vi "Close References.vi"(8 "error in":errorcluster, 11 "IProject Manager in":refnum<class "Mock IProject Manager.lvclass">) -> (0 "error out":errorcluster, 3 "IProject Manager out":refnum<class "Mock IProject Manager.lvclass">)   [LabVIEW 2026, in "Mock IProject Manager.lvclass"]
doc: "Close all project references."
uses:
  Mock IProject Manager.lvclass
  C:/Program Files/National Instruments/LabVIEW 2026/vi.lib/Astemes/LMock/Mock.lvclass
  <vilib>/Astemes/LMock/Mock.lvclass
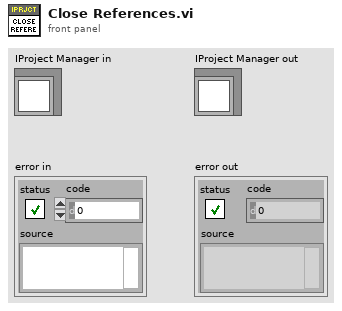
[diagram p1: front panel]
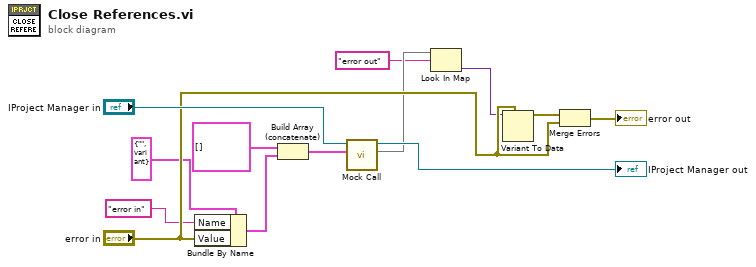
[diagram p0: block diagram]
diagram:
  n1 = Bundle By Name(cluster=cluster{"Name":string, "Value":variant} {"Name"="", "Value"=variant} ("element"), "Name"="error in", "Value"="error in") -> (w1:cluster{"Name":string, "Value":variant})
  n2 = Build Array (concatenate)(cluster{"Name":string, "Value":variant}[] [] ("Control Values"), w1) -> (w10:cluster{"Name":string, "Value":variant}[])
  n3 = call <vilib>:"Mock Call.vi"("Control Values"=w10, "Mock In"="IProject Manager in") -> ("Return Values"=w8:map{string, variant}, "Mock Out"=→"IProject Manager out":refnum<class "Mock IProject Manager.lvclass">)  [unwired: 8 in]
  n4 = Look In Map(map=w8, key="error out") -> (value=w6:variant)  [unwired: 1 in, 1 out]
  n5 = Variant To Data(type="error in", Variant=w6) -> (data=w5:errorcluster)  [unwired: 1 in, 1 out]
  n6 = Merge Errors(w5, "error in") -> (→"error out":errorcluster)
